vi "Read Double Direct.vi"(8 "error in (no error)":errorcluster, 11 "CIFTag in":refnum<class "CIF_Iceoryx_Chn_Double.lvclass">) -> (0 "error out":errorcluster, 2 "Data":dbl, 3 "CIFTag out":refnum<class "CIF_Iceoryx_Chn_Double.lvclass">)   [LabVIEW 2021, in "CIF_Iceoryx_Chn_Double.lvclass"]
uses:
  CIF_Iceoryx_Chn_Double.lvclass
  D:/dev/Packages/CIF_Channels_Core/src/Iceorxy_Channels/CIF_Iceoryx_BB/CIF_Iceoryx_BB.lvclass
  D:/dev/Packages/CIF_Channels_Core/src/CIFChannels/CIFChannels.lvclass
  CIF_Iceoryx_BB/CIF_Iceoryx_BB.lvclass/CIF_Iceoryx_BB.ctl
  CIFChannels/CIFChannels.lvclass/CIFChannels.ctl
  ChannelCommon/typedef/Channel State.ctl
  ChannelCommon/typedef/Direction.ctl
  CIF_Iceoryx_Chn_Double.lvclass/CIF_Iceoryx_Chn_Double.ctl
  e9c5801a-3ed8-4028-afd6-45613173f8eb.vi
  CIF_Iceoryx_BB/Accessors/Read Reader Reference.vi
  CIFChannels/Accessors/Read Tag Forced.vi
  CIFChannels/Accessors/Read Channel State.vi
  CIFChannels/Accessors/Read Direction.vi
  <vilib>/CIF Foundation/CIF Iceoryx/SubVIs/Get Path.vi
  <vilib>/CIF Foundation/CIF Iceoryx/SubVIs/Convert Error.vi
  <vilib>/CIF Foundation/CIF Iceoryx/Refnum/BB Reader from Refnum.vi
  <vilib>/CIF Foundation/CIF Iceoryx/SubVIs/Convert Error Core.vi
  ChannelCommon/ChannelCommon.lvlib
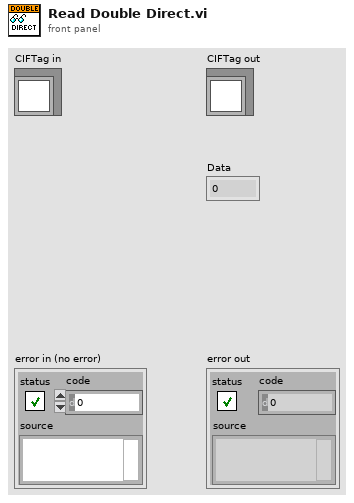
[diagram p1: front panel]
types:
  T1 = typedef "ChannelCommon.lvlib/Channel State.ctl" = enum8{"Creating", "Disconnected", "Connecting", "Connected", "Destroyed"}
  T2 = typedef "ChannelCommon.lvlib/Direction.ctl" = enum8{"Publisher", "Subscriber"}
  T3 = typedef "Iceoryx.lvlib/BB Reader Refnum.ctl" = cluster{"refnum":u64, "BB Reader":enum8{"bb_reader"}}
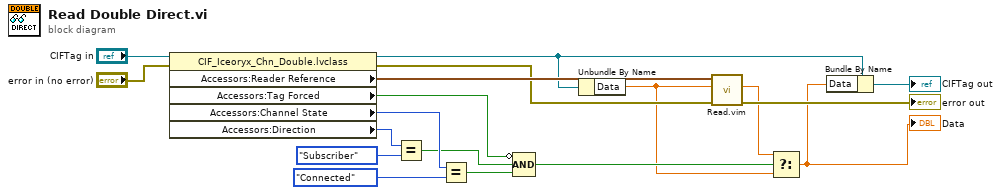
[diagram p0: block diagram]
diagram:
  n1 = property class="CIF_Iceoryx_Chn_Double.lvclass"(reference="CIFTag in", error in="error in (no error)") -> (reference out=w9:refnum<class "CIF_Iceoryx_Chn_Double.lvclass">, error out=w8:errorcluster, "Accessors:Reader Reference"=w10:T3, "Accessors:Tag Forced"=w5:bool, "Accessors:Channel State"=w13:T1, "Accessors:Direction"=w12:T2)
  n2 = Equal?(x=w12, y=Direction."Subscriber") -> (x = y?=w7:bool)
  n3 = Equal?(x=w13, y=Channel_State."Connected") -> (x = y?=w6:bool)
  n4 = Compound Arithmetic op=AND(invert w5, w7, w6) -> (w4:bool)
  n5 = Unbundle By Name(w9) -> ("Data"=w1:dbl)
  n6 = call "Read.vim"("error in (no error)"=w8, "Data In"=w1, "Reader Reference"=w10) -> ("error out"=→"error out":errorcluster, "Data Out"=w2:dbl)  [unwired: 6 in, 1 out]
  n7 = Select(t=w2, s=w4, f=w1) -> (s? t:f=w3:dbl)
  "Data" <- w3
  n8 = Bundle By Name(cluster=w9, "Data"=w3) -> (→"CIFTag out":refnum<class "CIF_Iceoryx_Chn_Double.lvclass">)
